vi "Max Plot Number--constant.vi"() -> (3 "Numeric":i32)   [LabVIEW 2020, in "Data Viewer.lvlib"]
uses:
  Data Viewer.lvlib
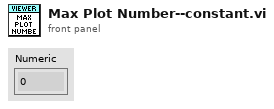
[diagram p1: front panel]
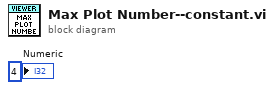
[diagram p0: block diagram]
diagram:
  "Numeric" <- 4
